vi "CSE - Open Callback VI Reference.vi"(6 "Save w/o diagram (F)":bool, 8 "error in":errorcluster, 9 "Window Title":string, 10 "Callback VI Path":path, 11 "CSE RefNum":T1) -> (0 "error out":errorcluster, 2 "Callback VI RefNum":T2, 3 "dup CSE RefNum":T1)   [LabVIEW 2021]
doc: "This VI opens a VI reference to a CSE Callback VI, prepares it for execution, and saves its path for further use. Refer to the VI help for more details.\n\nCallback VI path is used to open a reference to a Callback VI and pass it to CSE instance executing a script called from the initial script. This way, all CSE instances involved in a call chain of the top-level script will use the same Callback VI (but different instances of it if it's either a VI Template or a reentrant VI).\n\n<b>CSE RefNum</b> must contain a reference to a CSE instance context.\n\n::: CalcExpress Toolkit :::\nCopyright (c) 2000-2026 Konstantin Shifershteyn. All rights reserved."
uses:
  CSE Callback VI RefNum.ctl
  CSE Instance RefNum.ctl
panel:
  in  "Callback VI RefNum Template":T2
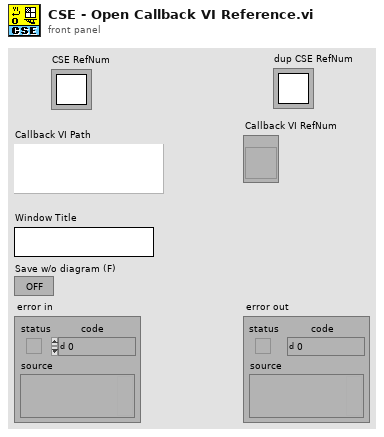
[diagram p1: front panel]
types:
  T1 = typedef "CSE Instance RefNum.ctl" = refnum<k1>
  T2 = typedef "CSE Callback VI RefNum.ctl" = refnum<vi>
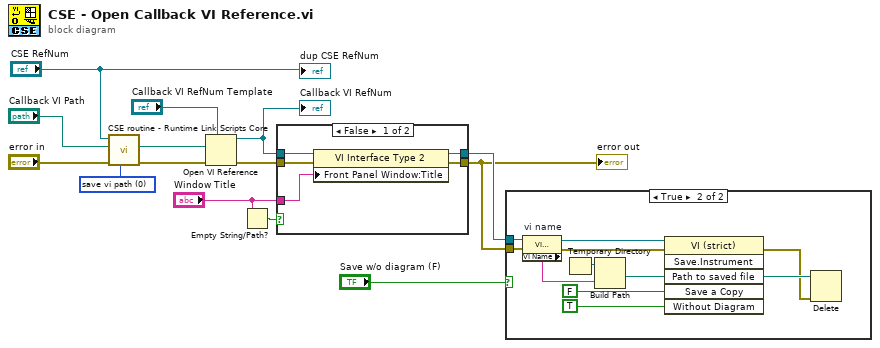
[diagram p0: block diagram]
diagram:
  w3 = 0 items=["save vi path", "link to caller", "delink of caller", "call-chain info"] ("action")
  n1 = call "CSE routine - Runtime Link Scripts Core.vi"("action"=w3, "error in"="error in", "Callback VI Path"="Callback VI Path", "CSE RefNum"="CSE RefNum") -> ("error out"=w12:errorcluster, "Callback VI Path out"=w11:path)  [unwired: 2 in, 4 out]
  n2 = Open VI Reference(type specifier VI Refnum (for type only)="Callback VI RefNum Template", vi path=w11, error in (no error)=w12) -> (vi reference=w7:T2, error out=w8:errorcluster)  [unwired: 3 in]
  "Callback VI RefNum" <- w7
  n3 = Empty String/Path?(string/path="Window Title") -> (empty?=w2:bool)
  n4 = case shown="False" w2 {
    tunnel: w7 -> [w19 w20]
    tunnel: w8 -> [w18 w21]
    tunnel: [w17 w21] -> w5
    tunnel: [w16 w20] -> w6
    tunnel: "Window Title" -> [w15 _]
    frame False {
      n5 = property class="VI Interface Type 2"(reference=w19, error in=w18, "Front Panel Window:Title"=w15) -> (reference out=w16:T2, error out=w17:errorcluster)
    }
    frame True {
    }
  }
  "error out" <- w5
  n6 = case shown="True" "Save w/o diagram (F)" {
    tunnel: w6 -> [_ w26]
    tunnel: w5 -> [_ w22]
    frame False {
    }
    frame True {
      n7 = property on="vi name" class="VI (strict)"(reference=w26, error in=w22) -> (reference out=w28:T2, error out=w27:errorcluster, "VI Name"=w29:string)
      n8 = Temporary Directory() -> (w31:path)
      n9 = Build Path(base path=w31, name or relative path=w29) -> (appended path=w30:path)
      n10 = invoke class="VI (strict)" method="Save.Instrument"(reference=w28, error in=w27, "Path to saved file"=w30, "Save a Copy"=FALSE, "Without Diagram"=TRUE) -> (error out=w23:errorcluster)  [unwired: 1 in, 5 out]
      n11 = Delete(path (use dialog)=w30, error in=w23) -> ()  [unwired: 3 in, 3 out]
    }
  }
  "dup CSE RefNum" <- "CSE RefNum"
